vi "CANSUB Write Xnet Frames.vi"(8 "error in (no error)":errorcluster, 9 "nBufferSize":i32, 10 "pBuffer":u8[](array[numeric])=array[4097 elements], 11 "nClientID":i16) -> (0 "error out":errorcluster, 2 "function return":i32, 3 "pFrameCount":i32)   [LabVIEW 2020, in "cansub_rp1210.lvlib"]
doc: "long __stdcall CANSUB_WriteXnetFrames(short nClientID, const unsigned char pBuffer[], long nBufferSize, long *pFrameCount);"
uses:
  cansub_rp1210.lvlib
  cansub_lv64.dll
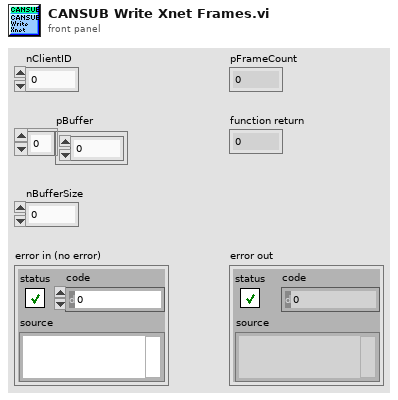
[diagram p1: front panel]
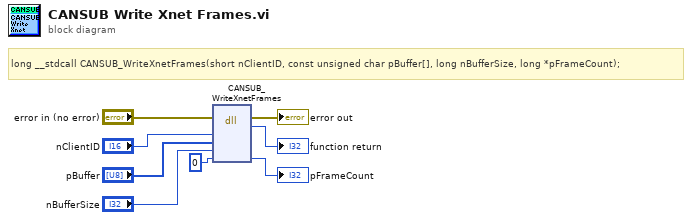
[diagram p0: block diagram]
diagram:
  # "long __stdcall CANSUB_WriteXnetFrames(short nClientID, const unsigned char pBuffer[], long nBufferSize, long *pFrameCount);"
  n1 = dll-call lib="C:/cansub-lv/library/cansub_lv*.*" fn="CANSUB_WriteXnetFrames"(error in="error in (no error)", "nClientID"="nClientID", "pBuffer"="pBuffer", "nBufferSize"="nBufferSize", "pFrameCount"=0) -> (error out=→"error out":errorcluster, "return type"=→"function return":i32, "pFrameCount"=→"pFrameCount":i32)  [unwired: 5 in, 1 out]
